vi "Test_2.vi"() -> ()   [LabVIEW 2024]
panel:
  out "Number":i32
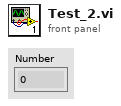
[diagram p1: front panel]
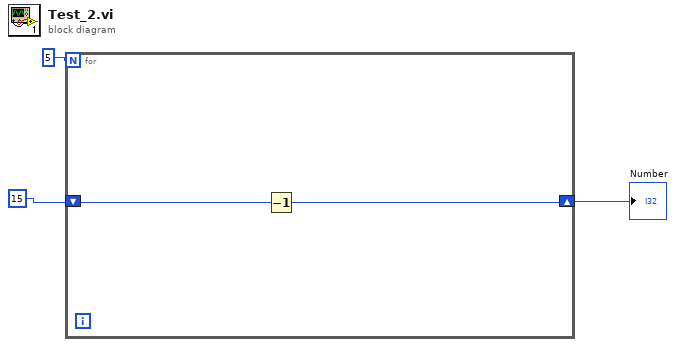
[diagram p0: block diagram]
diagram:
  n1 = for {
    N: 5 -> [_]
    shift-right: [w4] -> w1
    shift-left: 15 -> [w5]
    n2 = Decrement(x=w5) -> (x-1=w4:i32)
  }
  "Number" <- w1
